vi "OwnFile20261012_Native_AddConstantFromTypedef.vi"() -> ()   [LabVIEW 2024]
panel:
  out "error out":errorcluster caption="错误输出"
  out "terminal_id":u32
  in  "terminal_id type":u32
  out "constant_id":u32
  in  "constant_id type":u32
  in  "y":i16=100
  in  "x":i16=100
  in  "typedef_path":path
  in  "owner_diagram_id":u32
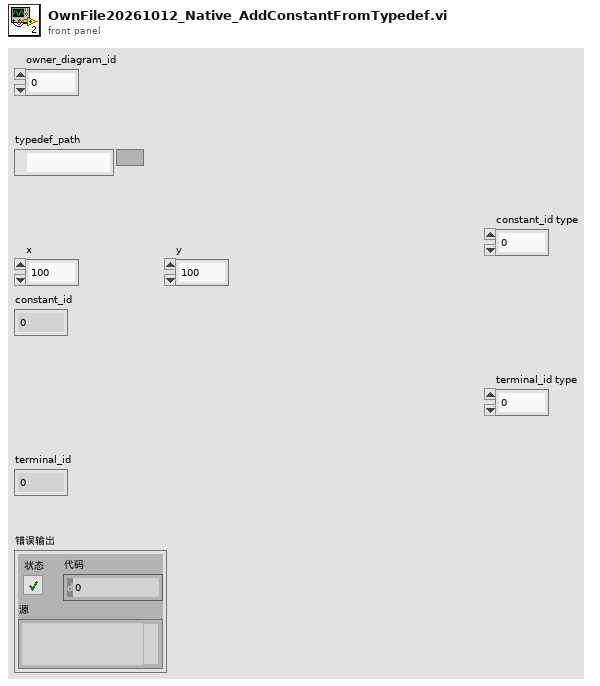
[diagram p1: front panel]
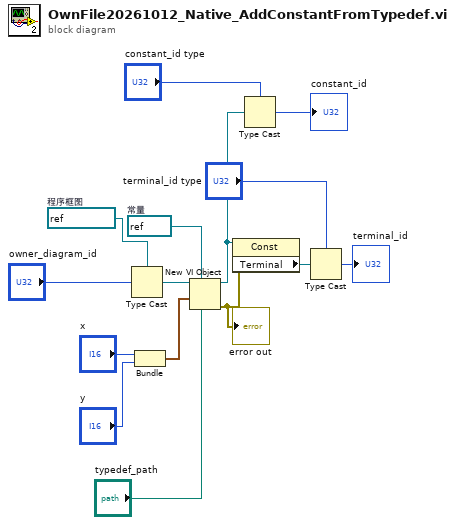
[diagram p0: block diagram]
diagram:
  w13 = refnum<vi> refnum  # 常量
  w14 = refnum<vi> refnum  # 程序框图
  n1 = Type Cast ("强制类型转换")(type=w14, x="owner_diagram_id") -> (*(type *) &x=w12:refnum<vi>)
  n2 = Bundle ("捆绑")("x"="x", "y"="y") -> (w8:cluster{"x":i16, "y":i16})  [unwired: 1 in]
  n3 = New VI Object ("新建VI对象")(vi object class=w13, owner refnum=w12, position/next to=w8, 6:"typedef_path") -> (object refnum=w7:refnum<vi>, 0:w1:errorcluster)  [unwired: 4 in]
  "error out" <- w1
  n4 = property on="属性节点" class="Const"(reference=w7, error in=w1) -> ("Terminal"=w4:refnum<vi>)  [unwired: 2 out]
  n5 = Type Cast ("强制类型转换")(type="constant_id type", x=w7) -> (*(type *) &x=→"constant_id":u32)
  n6 = Type Cast ("强制类型转换")(type="terminal_id type", x=w4) -> (*(type *) &x=→"terminal_id":u32)
